vi "Initialize to Existing File.vi"() -> ()   [LabVIEW 2018]
uses:
  src/api/logger_class/Log Levels.ctl
  bc269cd9-d162-4013-a312-bd866d79ee19.vi
  src/api/configuration/handlers/file_handler/File Handler.lvclass
  C:/Users/Colin/Documents/software_projects/labview/glog/src/api/extension/formatting_handler_interface/Formatting Handler.lvclass
  src/api/logger_class/Log (Parts).vi
  src/api/logger_class/Logger.lvclass
panel:
  in  "Cleanup Directory on Finish?":bool
  in  "initial filename":string="logfile_testing_2026_05_13.log"
  in  "file name format":string="logfile_testing_%<%Y_%m_%d>T.log"
  out "error out":errorcluster
  in  "Stop":bool
  # "Locals"
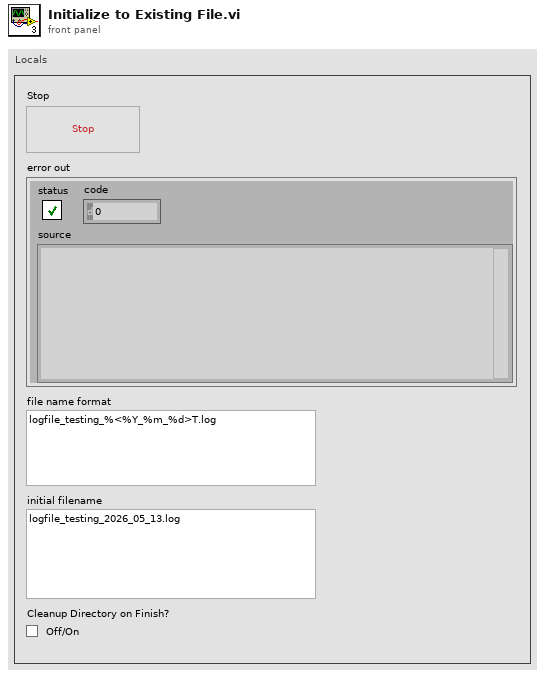
[diagram p1: front panel]
types:
  T1 = enum16{"open", "replace", "create", "open or create", "replace or create", "replace or create with confirmation"}
  T2 = typedef "GLog.lvlib/Logger.lvclass/Log Levels.ctl" = enum16{"Trace", "Debug", "Info", "Warning", "Error", "Critical"}
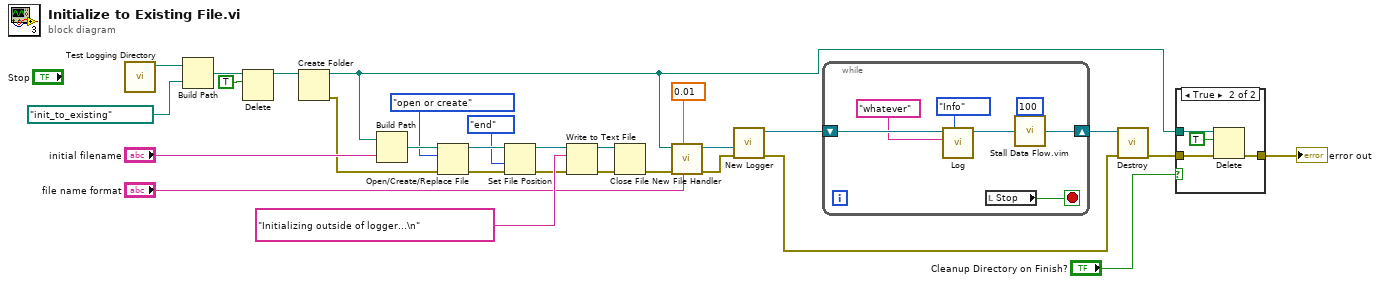
[diagram p0: block diagram]
diagram:
  n1 = call "Test Logging Directory.vi"() -> ("test logging directory"=w11:path)  [unwired: 11 in]
  n2 = Build Path(base path=w11, name or relative path=path "init_to_existing") -> (appended path=w9:path)
  n3 = Delete(path (use dialog)=w9, entire hierarchy (F)=TRUE) -> (deleted path=w4:path)  [unwired: 3 in, 2 out]
  n4 = Create Folder(path (use dialog)=w4) -> (created path=w3:path, error out=w2:errorcluster)  [unwired: 2 in, 1 out]
  n5 = Build Path(base path=w3, name or relative path="initial filename") -> (appended path=w26:path)
  n6 = Open/Create/Replace File(file path (use dialog)=w26, error in=w2, operation (0:open)=T1."open or create") -> (refnum out=w18:refnum<file>, error out=w16:errorcluster)  [unwired: 3 in, 1 out]
  n7 = Set File Position(refnum=w18, from (0:start)=enum16{"start", "end", "current"}."end", error in=w16) -> (refnum out=w19:refnum<file>, error out=w15:errorcluster)  [unwired: 1 in]
  n8 = Write to Text File(file (use dialog)=w19, text="Initializing outside of logger...\n", error in=w15) -> (refnum out=w23:refnum<file>, error out=w24:errorcluster)  [unwired: 1 in, 1 out]
  n9 = Close File(refnum=w23, error in=w24) -> (error out=w22:errorcluster)  [unwired: 1 out]
  n10 = call "New File Handler.vi"("file name format (\"logfile_%<%Y-%m-%d_%H-%M-%S>T.log\")"="file name format", "max file size [MB](50)"=0.01, "error in"=w22, "log directory (<app dir>/logs)"=w3) -> ("error out"=w21:errorcluster, "file handler"=w29:refnum<class "File Handler.lvclass">)  [unwired: 5 in, 1 out]
  n11 = call "New Logger.vi"("error in (no error)"=w21, "log handler (file handler)"=w29) -> ("error out"=w20:errorcluster, "logger"=w28:refnum<class "Logger.lvclass">)  [unwired: 8 in]
  n12 = while {
    shift-right: [w33] -> w27
    shift-left: w28 -> [w36]
    stop <- w31 stop-if-true
    n13 = call-poly "Log.vi"("log level"=Log_Levels."Info", "message"="whatever", "logger in"=w36) -> ("logger out"=w34:refnum<class "Logger.lvclass">)  [unwired: 8 in]
    n14 = local read "Stop"() -> (w31:bool)
    n15 = call "Stall Data Flow.vim"("value in"=w34, "milliseconds to wait"=u32 100) -> ("value out"=w33:refnum<class "Logger.lvclass">)  [unwired: 1 out]
  }
  n16 = call "Destroy.vi"("error in (no error)"=w20, "logger in"=w27) -> ("error out"=w7:errorcluster)  [unwired: 8 in, 1 out]
  n17 = case shown="True" "Cleanup Directory on Finish?" {
    tunnel: w7 -> [w37 w41]
    tunnel: [w37 w40] -> w6
    tunnel: w3 -> [_ w39]
    frame False {
    }
    frame True {
      n18 = Delete(path (use dialog)=w39, entire hierarchy (F)=TRUE, error in=w41) -> (error out=w40:errorcluster)  [unwired: 2 in, 2 out]
    }
  }
  "error out" <- w6
